vi "Autonomous Independent.vi"() -> ()   [LabVIEW 2015]
doc: "This VI is called when autonomous begins, and will automatically be terminated when autonomous ends. You can carry out timed or sensor driven robot movement independently without needing to return to the caller."
uses:
  <vilib>/Rock Robotics/WPI/Solenoid/WPI_SolenoidValue.ctl
  <vilib>/Rock Robotics/WPI/Utilities/WPI_GetSetVariantRefNum.vi
  <vilib>/Rock Robotics/Network Tables/NT Read String.vi
  <vilib>/Rock Robotics/Network Tables/NT Write Numeric Array.vi
  <vilib>/Rock Robotics/WPI/Solenoid/WPI_SolenoidSetEnum.vi
  <vilib>/Rock Robotics/WPI/RobotDrive/WPI_RobotDriveArcadeDrive_Standard(NoSaturation).vi
panel:
  in  "Compensation Arrière":dbl=-0.2 min=-1.0 max=1.0 step=0.05 format="%#_13g"
  in  "Enable ShakeUp":bool=TRUE
  in  "ShakeUp Delay":dbl=0.15000000000000002 min=0.0 max=2.0 step=0.05
  in  "Compensation Avant":dbl=-0.2 min=-1.0 max=1.0 step=0.05 format="%#_13g"
  in  "Temps":dbl=6.0 format="%#_13g"
  in  "Power":dbl=0.7000000000000002 min=0.0 max=1.0 step=0.05 format="%#_13g"
  # "Be sure to right-click and choose Data Operations>>Make Current Value default if you want to save the array values with the VI"
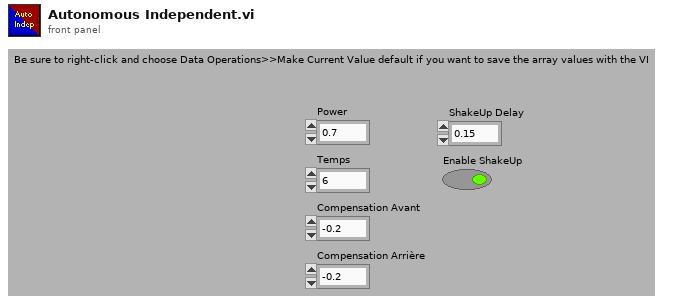
[diagram p1: front panel]
types:
  T1 = typedef "WPI_JoystickDevRef.ctl" = cluster{"Device":T2}
  T2 = typedef "WPI_JoystickDeviceEnum.ctl" = enum16{"USB 0", "USB 1", "USB 2", "USB 3", "USB 4", "USB 5"}
  T3 = typedef "WPI_SolenoidValue.ctl" = enum16{"Off", "On", "Forward", "Reverse"}
  T4 = typedef "WPI_SolenoidDevRef.ctl" = cluster{"DevStatus":errorcluster, "Pneumatics Control Module":u8, "Forward Solenoid Channel":T5, "Reverse Solenoid Channel":T5}
  T5 = typedef "WPI_SolenoidChannel.ctl" = enum8{"Solenoid 0", "Solenoid 1", "Solenoid 2", "Solenoid 3", "Solenoid 4", "Solenoid 5", "Solenoid 6", "Solenoid 7", "Invalid"}
  T6 = typedef "WPI_RobotDriveDevRef.ctl" = cluster{"DevStatus":errorcluster, "Motors[]":T7[], "Square Inputs":bool, "Max Output":dbl}
  T7 = typedef "WPI_MotorControlDeviceRef.ctl" = cluster{"DeviceStatus":errorcluster, "Type":T8, "PWM":cluster{"PWM Channel":T9, "DeadBand":T10}, "CAN":cluster{"Device Number":u8, "Control Mode":T11, "Semaphore":T12, "Max Vout":dbl, "TalonSRX Control Mode":T13}, "Invert":bool}
  T8 = typedef "WPI_MotorControlType.ctl" = enum16{"PWM", "CAN", "CANTalonSRX"}
  T9 = typedef "FPGA_DIOPWMChannel.ctl" = enum8{"PWM 0", "PWM 1", "PWM 2", "PWM 3", "PWM 4", "PWM 5", "PWM 6", "PWM 7", "PWM 8", "PWM 9", "PWM MXP 0", "PWM MXP 1", "PWM MXP 2", "PWM MXP 3", "PWM MXP 4", "PWM MXP 5", "PWM MXP 6", "PWM MXP 7", "PWM MXP 8", "PWM MXP 9", "Invalid"}
  T10 = typedef "WPI_PWMDeadband.ctl" = cluster{"Name":string, "maxPositivePwm":i32, "minPositivePwm":i32, "centerPwm":i32, "maxNegativePwm":i32, "minNegativePwm":i32, "angularRange":u16}
  T11 = typedef "WPI_CANJaguar_ControlMode.ctl" = enum8{"Percent VBus", "Current", "Speed", "Position", "Voltage"}
  T12 = typedef "Semaphore RefNum" = refnum<k1>
  T13 = typedef "WPI_CANTalonSRX_APIControlMode.ctl" = enum8{"Percent VBus", "Speed", "Position", "Slave", "Unchanged / Invalid", "Voltage Compensation", "Current", "Motion Profile"}
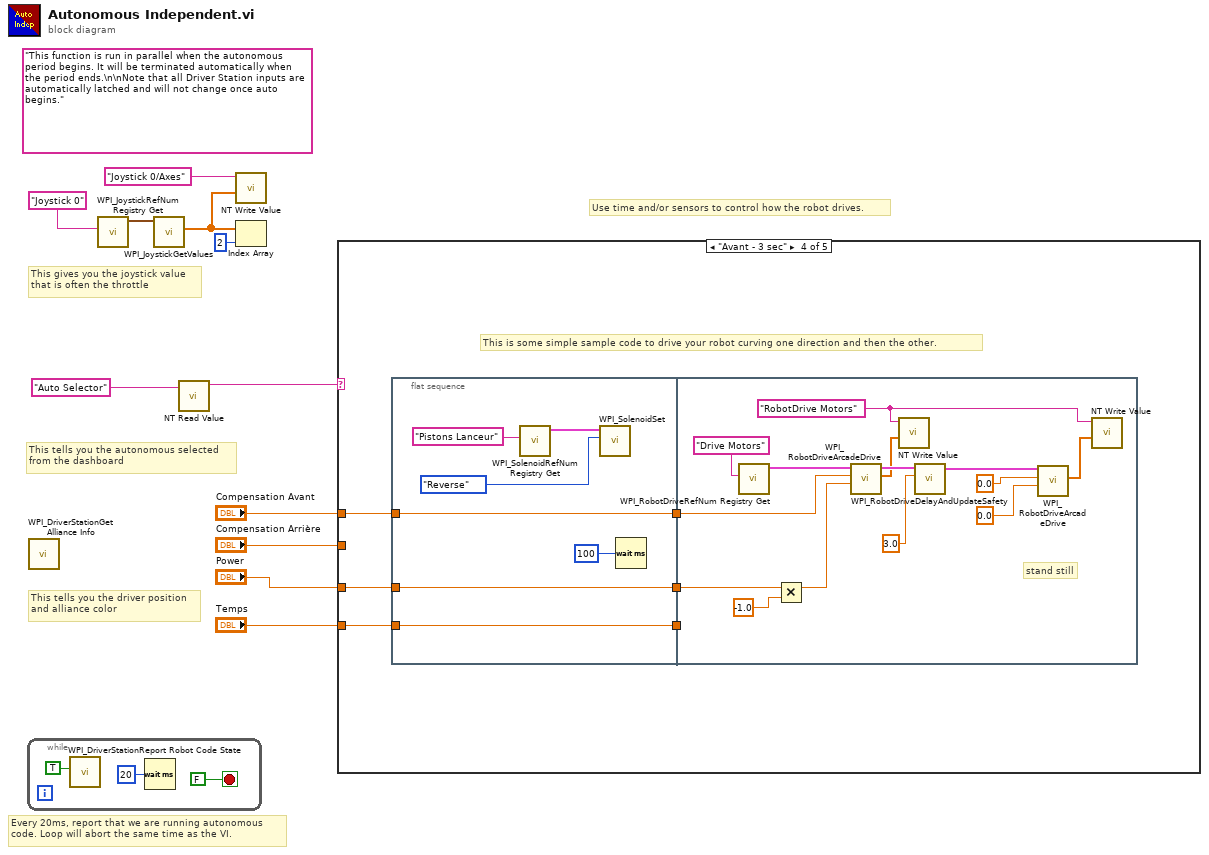
[diagram p0: block diagram]
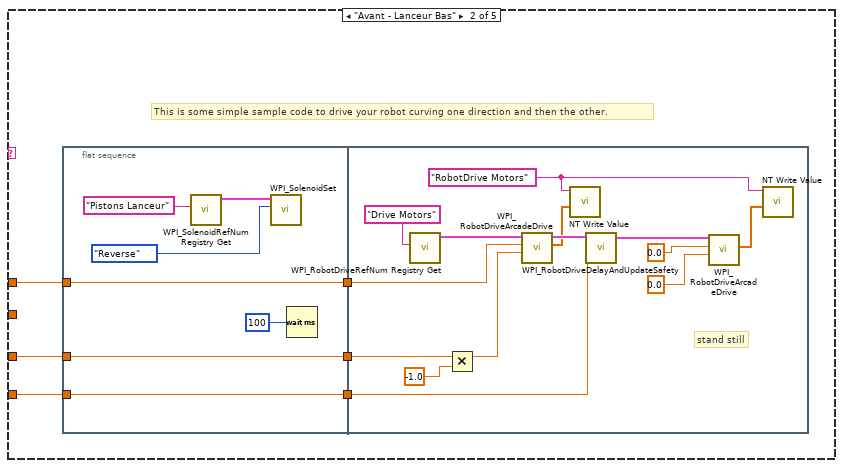
[diagram p3: hidden frame]
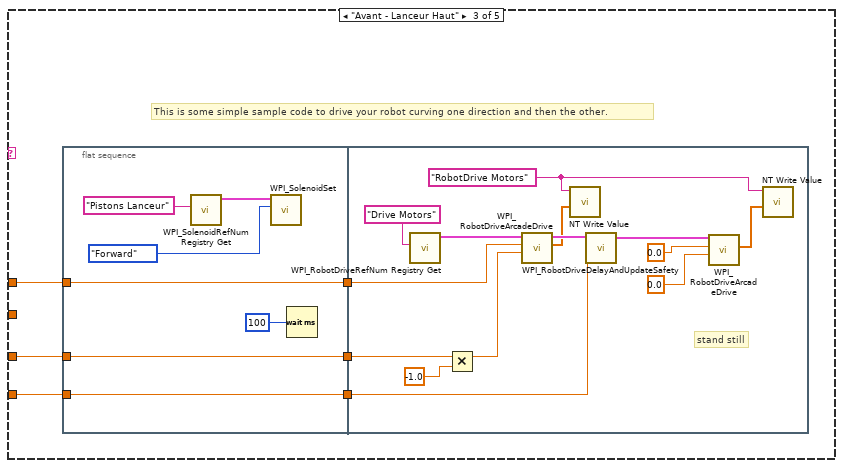
[diagram p4: hidden frame]
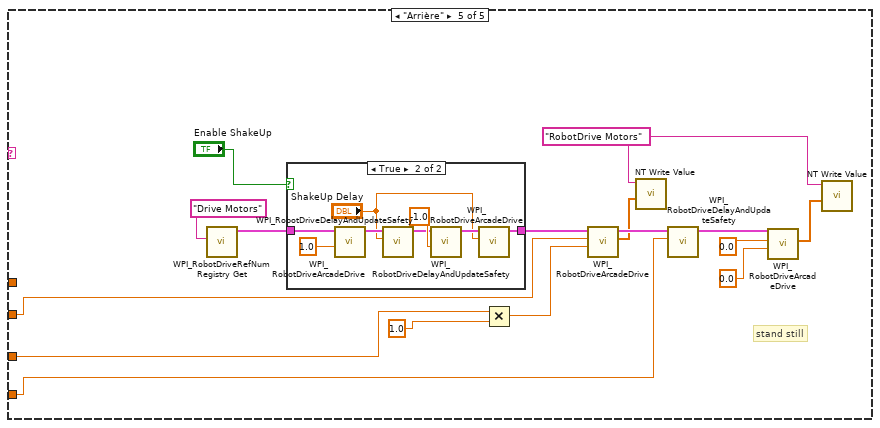
[diagram p5: hidden frame]
diagram:
  (unwired) "This function is run in parallel when the autonomous period begins. It will be terminated automatically when the period ends.\n\nNote that all Driver Station inputs are automatically latched and will not change once auto begins."
  # "This tells you the autonomous selected\nfrom the dashboard"
  # "Every 20ms, report that we are running autonomous\ncode. Loop will abort the same time as the VI."
  # "This gives you the joystick value\nthat is often the throttle"
  # "Use time and/or sensors to control how the robot drives."
  # "This tells you the driver position\nand alliance color"
  n1 = while {
    stop <- FALSE stop-if-true
    n2 = call <vilib>:"WPI_DriverStationReport Robot Code State.vi"("Autonomous"=TRUE) -> ()  [unwired: 10 in, 1 out]
    n3 = Wait (ms)(milliseconds to wait=u32 20) -> ()  [unwired: 1 out]
  }
  n4 = call <vilib>:"WPI_DriverStationGet Alliance Info.vi"() -> ()  [unwired: 12 out]
  n5 = call <vilib>:"WPI_JoystickRefNum Registry Get.vi"("refnum name"="Joystick 0") -> ("JoystickDevRef"=w10:T1)  [unwired: 1 in, 9 out]
  n6 = call <vilib>:"WPI_JoystickGetValues.vi"("JoystickDevRef"=w10) -> ("Axes"=w7:dbl[])  [unwired: 6 in, 4 out]
  n7 = call-poly <vilib>:"NT Read Value.vi"("Name"="Auto Selector") -> ("String"=w5:string)  [unwired: 9 in, 1 out]
  n8 = call-poly <vilib>:"NT Write Value.vi"("Numeric Array"=w7, "Name"="Joystick 0/Axes") -> ()  [unwired: 9 in, 1 out]
  n9 = Index Array(array=w7, index=2) -> ()  [unwired: 1 out]
  n10 = case shown="\"Avant - 3 sec\"" w5 {
    tunnel: "Compensation Avant" -> [_ w20 w47 w74 _]
    tunnel: "Power" -> [_ w19 w46 w73 w103]
    tunnel: "Temps" -> [_ w18 w45 w72 w102]
    tunnel: "Compensation Arrière" -> [_ _ _ _ w96]
    frame Default {
      # "You can put your main auto here, or you can right-click on the case and make any\nother frame be the default case."
      # "This is the frame that will execute if no selection is made, or if it is not recognized"
    }
    frame "Avant - Lanceur Bas" {
      # "This is some simple sample code to drive your robot curving one direction and then the other."
      n11 = flat-sequence {
        tunnel: w18 -> [w25]
        tunnel: w19 -> [w26]
        tunnel: w20 -> [w27]
        tunnel: [w27] -> w17
        tunnel: [w26] -> w16
        tunnel: [w25] -> w15
        tunnel: w17 -> [w31]
        tunnel: w16 -> [w30]
        tunnel: w15 -> [w29]
        frame #0 {
          n12 = call <vilib>:"WPI_SolenoidRefNum Registry Get.vi"("refnum name"="Pistons Lanceur") -> ("SolenoidDevRef"=w22:T4)  [unwired: 9 in, 1 out]
          n13 = call-poly <vilib>:"WPI_SolenoidSet.vi"("Value"=WPI_SolenoidValue."Reverse", "SolenoidDevRef"=w22) -> ()  [unwired: 8 in, 2 out]
          n14 = Wait (ms)(milliseconds to wait=u32 100) -> ()  [unwired: 1 out]
        }
        frame #1 {
          w32 = "RobotDrive Motors" ("Name")
          # "stand still"
          n15 = call <vilib>:"WPI_RobotDriveRefNum Registry Get.vi"("refnum name"="Drive Motors") -> ("RobotDriveDevRef"=w41:T6)  [unwired: 1 in, 9 out]
          n16 = Multiply(x=w30, y=-1.0) -> (x*y=w34:dbl)
          n17 = call-poly <vilib>:"WPI_RobotDriveArcadeDrive.vi"("Y axis value"=w34, "X axis value"=w31, "RobotDriveDevRef"=w41) -> ("Motor Values"=w35:dbl[], "RobotDriveDevRef"=w39:T6)  [unwired: 1 in, 6 out]
          n18 = call-poly <vilib>:"NT Write Value.vi"("Numeric Array"=w35, "Name"=w32) -> ()  [unwired: 9 in, 1 out]
          n19 = call <vilib>:"WPI_RobotDriveDelayAndUpdateSafety.vi"("Delay (s)"=w29, "RobotDriveDevRef"=w39) -> ("RobotDriveDevRef 2"=w33:T6)  [unwired: 8 in, 1 out]
          n20 = call-poly <vilib>:"WPI_RobotDriveArcadeDrive.vi"("Y axis value"=0.0 ("X axis value"), "X axis value"=0.0, "RobotDriveDevRef"=w33) -> ("Motor Values"=w36:dbl[])  [unwired: 1 in, 7 out]
          n21 = call-poly <vilib>:"NT Write Value.vi"("Numeric Array"=w36, "Name"=w32) -> ()  [unwired: 9 in, 1 out]
        }
      }
    }
    frame "Avant - Lanceur Haut" {
      # "This is some simple sample code to drive your robot curving one direction and then the other."
      n22 = flat-sequence {
        tunnel: w45 -> [w52]
        tunnel: w46 -> [w53]
        tunnel: w47 -> [w54]
        tunnel: [w54] -> w44
        tunnel: [w53] -> w43
        tunnel: [w52] -> w42
        tunnel: w44 -> [w58]
        tunnel: w43 -> [w57]
        tunnel: w42 -> [w56]
        frame #0 {
          n23 = call <vilib>:"WPI_SolenoidRefNum Registry Get.vi"("refnum name"="Pistons Lanceur") -> ("SolenoidDevRef"=w49:T4)  [unwired: 9 in, 1 out]
          n24 = call-poly <vilib>:"WPI_SolenoidSet.vi"("Value"=WPI_SolenoidValue."Forward", "SolenoidDevRef"=w49) -> ()  [unwired: 8 in, 2 out]
          n25 = Wait (ms)(milliseconds to wait=u32 100) -> ()  [unwired: 1 out]
        }
        frame #1 {
          w59 = "RobotDrive Motors" ("Name")
          # "stand still"
          n26 = call <vilib>:"WPI_RobotDriveRefNum Registry Get.vi"("refnum name"="Drive Motors") -> ("RobotDriveDevRef"=w68:T6)  [unwired: 1 in, 9 out]
          n27 = Multiply(x=w57, y=-1.0) -> (x*y=w61:dbl)
          n28 = call-poly <vilib>:"WPI_RobotDriveArcadeDrive.vi"("Y axis value"=w61, "X axis value"=w58, "RobotDriveDevRef"=w68) -> ("Motor Values"=w62:dbl[], "RobotDriveDevRef"=w66:T6)  [unwired: 1 in, 6 out]
          n29 = call-poly <vilib>:"NT Write Value.vi"("Numeric Array"=w62, "Name"=w59) -> ()  [unwired: 9 in, 1 out]
          n30 = call <vilib>:"WPI_RobotDriveDelayAndUpdateSafety.vi"("Delay (s)"=w56, "RobotDriveDevRef"=w66) -> ("RobotDriveDevRef 2"=w60:T6)  [unwired: 8 in, 1 out]
          n31 = call-poly <vilib>:"WPI_RobotDriveArcadeDrive.vi"("Y axis value"=0.0 ("X axis value"), "X axis value"=0.0, "RobotDriveDevRef"=w60) -> ("Motor Values"=w63:dbl[])  [unwired: 1 in, 7 out]
          n32 = call-poly <vilib>:"NT Write Value.vi"("Numeric Array"=w63, "Name"=w59) -> ()  [unwired: 9 in, 1 out]
        }
      }
    }
    frame "Avant - 3 sec" {
      # "This is some simple sample code to drive your robot curving one direction and then the other."
      n33 = flat-sequence {
        tunnel: w72 -> [w79]
        tunnel: w73 -> [w80]
        tunnel: w74 -> [w81]
        tunnel: [w81] -> w71
        tunnel: [w80] -> w70
        tunnel: [w79] -> w69
        tunnel: w71 -> [w85]
        tunnel: w70 -> [w84]
        tunnel: w69 -> [_]
        frame #0 {
          n34 = call <vilib>:"WPI_SolenoidRefNum Registry Get.vi"("refnum name"="Pistons Lanceur") -> ("SolenoidDevRef"=w76:T4)  [unwired: 9 in, 1 out]
          n35 = call-poly <vilib>:"WPI_SolenoidSet.vi"("Value"=WPI_SolenoidValue."Reverse", "SolenoidDevRef"=w76) -> ()  [unwired: 8 in, 2 out]
          n36 = Wait (ms)(milliseconds to wait=u32 100) -> ()  [unwired: 1 out]
        }
        frame #1 {
          w86 = "RobotDrive Motors" ("Name")
          # "stand still"
          n37 = call <vilib>:"WPI_RobotDriveRefNum Registry Get.vi"("refnum name"="Drive Motors") -> ("RobotDriveDevRef"=w95:T6)  [unwired: 1 in, 9 out]
          n38 = Multiply(x=w84, y=-1.0) -> (x*y=w88:dbl)
          n39 = call-poly <vilib>:"WPI_RobotDriveArcadeDrive.vi"("Y axis value"=w88, "X axis value"=w85, "RobotDriveDevRef"=w95) -> ("Motor Values"=w89:dbl[], "RobotDriveDevRef"=w93:T6)  [unwired: 1 in, 6 out]
          n40 = call-poly <vilib>:"NT Write Value.vi"("Numeric Array"=w89, "Name"=w86) -> ()  [unwired: 9 in, 1 out]
          n41 = call <vilib>:"WPI_RobotDriveDelayAndUpdateSafety.vi"("Delay (s)"=3.0, "RobotDriveDevRef"=w93) -> ("RobotDriveDevRef 2"=w87:T6)  [unwired: 8 in, 1 out]
          n42 = call-poly <vilib>:"WPI_RobotDriveArcadeDrive.vi"("Y axis value"=0.0 ("X axis value"), "X axis value"=0.0, "RobotDriveDevRef"=w87) -> ("Motor Values"=w90:dbl[])  [unwired: 1 in, 7 out]
          n43 = call-poly <vilib>:"NT Write Value.vi"("Numeric Array"=w90, "Name"=w86) -> ()  [unwired: 9 in, 1 out]
        }
      }
    }
    frame "Arrière" {
      w104 = "RobotDrive Motors" ("Name")
      # "stand still"
      n44 = call <vilib>:"WPI_RobotDriveRefNum Registry Get.vi"("refnum name"="Drive Motors") -> ("RobotDriveDevRef"=w99:T6)  [unwired: 1 in, 9 out]
      n45 = case shown="True" "Enable ShakeUp" {
        tunnel: [w112 w114] -> w100
        tunnel: w99 -> [w112 w113]
        frame False {
        }
        frame True {
          n46 = call-poly <vilib>:"WPI_RobotDriveArcadeDrive.vi"("Y axis value"=1.0, "RobotDriveDevRef"=w113) -> ("RobotDriveDevRef"=w119:T6)  [unwired: 2 in, 7 out]
          n47 = call <vilib>:"WPI_RobotDriveDelayAndUpdateSafety.vi"("Delay (s)"="ShakeUp Delay", "RobotDriveDevRef"=w119) -> ("RobotDriveDevRef 2"=w116:T6)  [unwired: 8 in, 1 out]
          n48 = call-poly <vilib>:"WPI_RobotDriveArcadeDrive.vi"("Y axis value"=-1.0, "RobotDriveDevRef"=w116) -> ("RobotDriveDevRef"=w118:T6)  [unwired: 2 in, 7 out]
          n49 = call <vilib>:"WPI_RobotDriveDelayAndUpdateSafety.vi"("Delay (s)"="ShakeUp Delay", "RobotDriveDevRef"=w118) -> ("RobotDriveDevRef 2"=w114:T6)  [unwired: 8 in, 1 out]
        }
      }
      n50 = Multiply(x=w103, y=1.0 ("t")) -> (x*y=w105:dbl)
      n51 = call-poly <vilib>:"WPI_RobotDriveArcadeDrive.vi"("Y axis value"=w105, "X axis value"=w96, "RobotDriveDevRef"=w100) -> ("Motor Values"=w106:dbl[], "RobotDriveDevRef"=w110:T6)  [unwired: 1 in, 6 out]
      n52 = call-poly <vilib>:"NT Write Value.vi"("Numeric Array"=w106, "Name"=w104) -> ()  [unwired: 9 in, 1 out]
      n53 = call <vilib>:"WPI_RobotDriveDelayAndUpdateSafety.vi"("Delay (s)"=w102, "RobotDriveDevRef"=w110) -> ("RobotDriveDevRef 2"=w101:T6)  [unwired: 8 in, 1 out]
      n54 = call-poly <vilib>:"WPI_RobotDriveArcadeDrive.vi"("Y axis value"=0.0 ("X axis value"), "X axis value"=0.0, "RobotDriveDevRef"=w101) -> ("Motor Values"=w107:dbl[])  [unwired: 1 in, 7 out]
      n55 = call-poly <vilib>:"NT Write Value.vi"("Numeric Array"=w107, "Name"=w104) -> ()  [unwired: 9 in, 1 out]
    }
  }
